vi "VIH ProjFile - Path Array - Read.vi"(8 "error in":errorcluster, 10 "Property Name":string, 11 "XML Parent Item":refnum<k20>) -> (0 "error out":errorcluster, 1 "Files":path[](array[path]), 3 "dup XML Parent Item":refnum<k20>)   [LabVIEW 2014]
doc: "::: VI Helpeks :::\nCopyright (c) 2000-2026 Konstantin Shifershteyn. All rights reserved."
uses:
  <vilib>/xml/Close Reference(Node).vi
  <vilib>/xml/NI_XML.lvlib
panel:
  # "VI Helpeks\nCopyright (c) 2012-2026 Konstantin Shifershteyn"
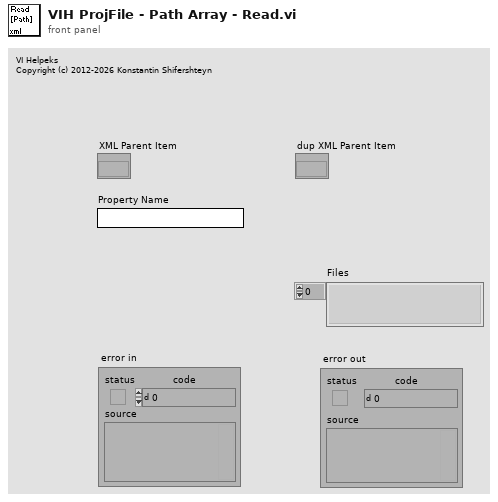
[diagram p1: front panel]
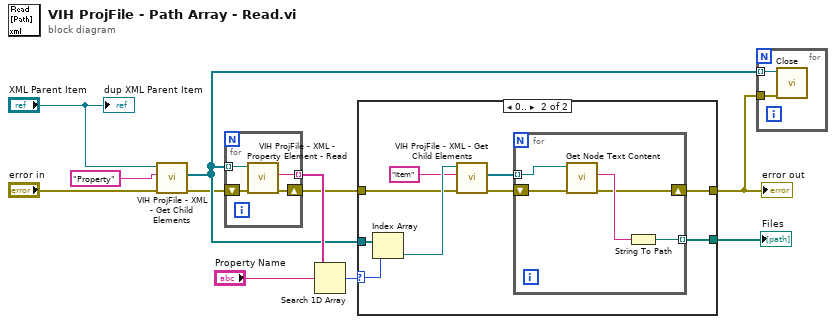
[diagram p0: block diagram]
diagram:
  n1 = call "VIH ProjFile - XML - Get Child Elements.vi"("error in"="error in", "Tag Name"="Property", "XML Parent Item"="XML Parent Item") -> ("error out"=w4:errorcluster, "Array of Elements"=w5:refnum<k20>[])  [unwired: 6 in, 1 out]
  n2 = for {
    tunnel: w5 -> [w15] mode=indexing
    shift-right: [w13] -> w9
    shift-left: w4 -> [w14]
    tunnel: [w12] -> w11 mode=indexing
    n3 = call "VIH ProjFile - XML - Property Element - Read.vi"("error in"=w14, "XML Node"=w15) -> ("error out"=w13:errorcluster, "Property Name"=w12:string)  [unwired: 6 in, 2 out]
  }
  n4 = Search 1D Array(1D array=w11, element="Property Name") -> (index of element=w10:i32)  [unwired: 1 in]
  n5 = case shown="0.." w10 {
    selector: w10 -> [_ w24]
    tunnel: [w16 w23] -> w7
    tunnel: w9 -> [w16 w17]
    tunnel: w5 -> [_ w25]
    tunnel: [_ w22] -> w8
    frame ..-1 {
    }
    frame 0.. {
      n6 = Index Array(array=w25, index=w24) -> (element=w19:refnum<k20>)
      n7 = call "VIH ProjFile - XML - Get Child Elements.vi"("error in"=w17, "Tag Name"="Item", "XML Parent Item"=w19) -> ("error out"=w20:errorcluster, "Array of Elements"=w21:refnum<k20>[])  [unwired: 6 in, 1 out]
      n8 = for {
        tunnel: w21 -> [w29] mode=indexing
        shift-right: [w26] -> w23
        shift-left: w20 -> [w27]
        tunnel: [w30] -> w22 mode=indexing
        n9 = call <vilib>:"Get Node Text Content.vi"("error in (no error)"=w27, "node in"=w29) -> ("error out"=w26:errorcluster, "node text"=w28:string)  [unwired: 7 in, 1 out]
        n10 = String To Path(string=w28) -> (path=w30:path)
      }
    }
  }
  "error out" <- w7
  "Files" <- w8
  n11 = for {
    tunnel: w5 -> [w32] mode=indexing
    tunnel: w7 -> [w31]
    n12 = call-poly <vilib>:"Close.vi"("error in (no error)"=w31, "node"=w32) -> ()  [unwired: 7 in, 1 out]
  }
  "dup XML Parent Item" <- "XML Parent Item"
